vi "Scanning_ESR.vi"() -> ()   [LabVIEW 2024]
panel:
  out "Direction Indicator":bool
  in  "Direction":bool
  out "Y Steps":i32
  out "Data 2":string[][](array[string])
  out "Unaveraged data 2":string[][](array[string])
  out "Data":string[][](array[string])
  out "Unaveraged data":string[][](array[string])
  in  "file path (use dialog) 2":path=path "C:/Users/Crawford Group/Desktop/Angelo/NMR/DATA/Unaveraged&TimeStamp.txt"
  in  "file path (use dialog)":path=path "C:/Users/Crawford Group/Desktop/Angelo/NMR/DATA/DATA.txt"
  out "error out 2":errorcluster
  out "error out":errorcluster
  in  "Up?":bool
  out "Number of X":i32
  in  "Step size mm  Y":dbl=0.0017
  in  "Y Motor":refnum<k7>(container)
  in  "Step size mm X":dbl=0.0098
  in  "X Motor":refnum<k7>(container)
  in  "Number of X steps":dbl=1.0
  in  "Sweeps?":i32=1
  # "Averaged"
  # "Unaveraged"
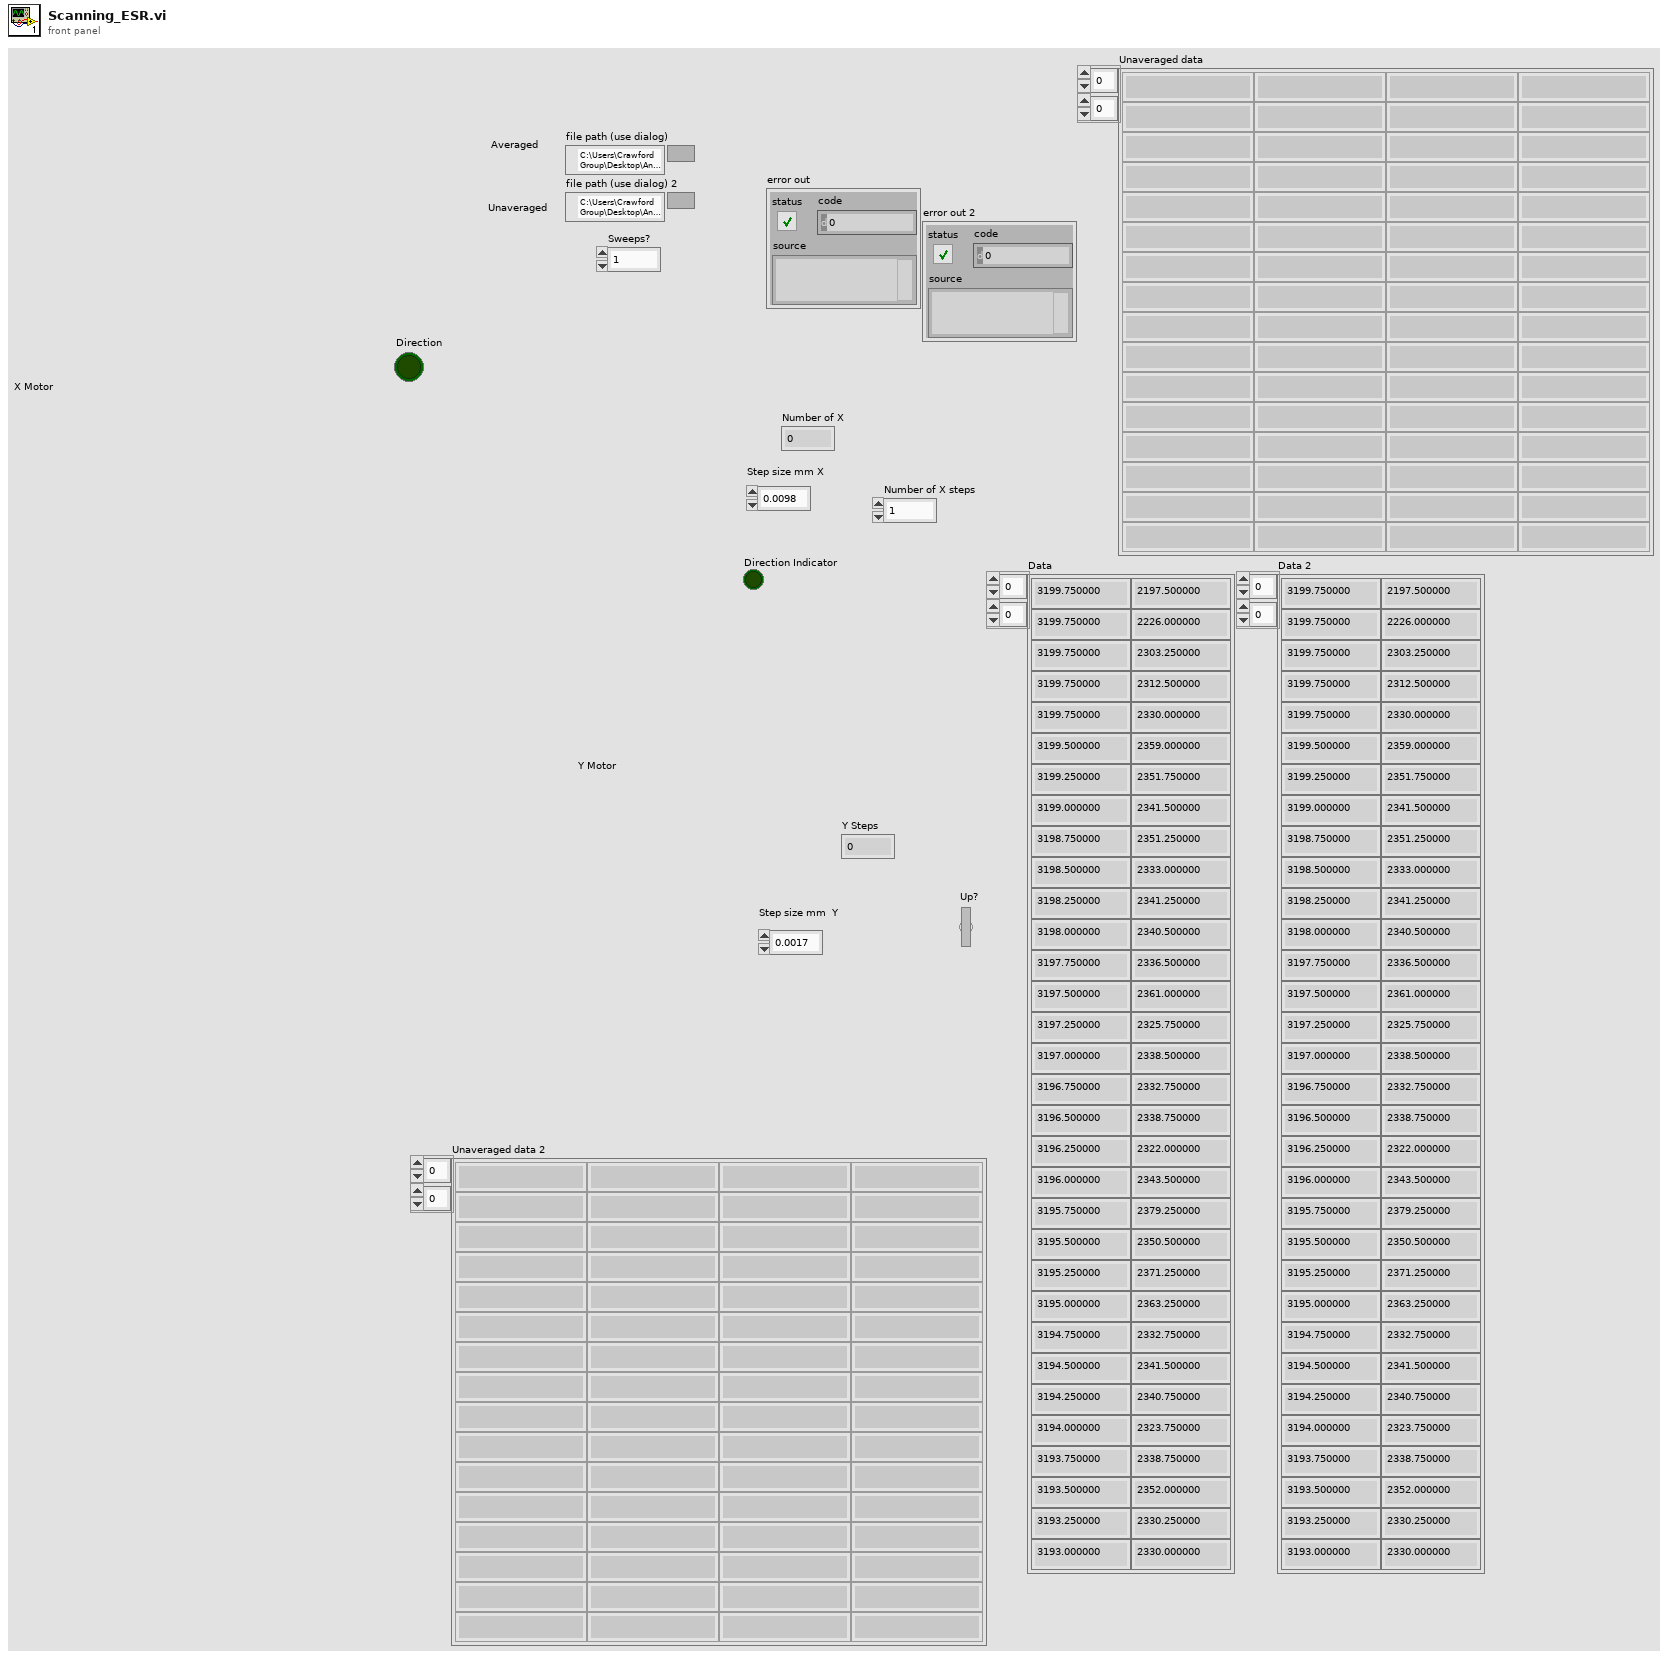
[diagram p1: front panel]
types:
  T1 = enum16{"open", "replace", "create", "open or create", "replace or create", "replace or create with confirmation"}
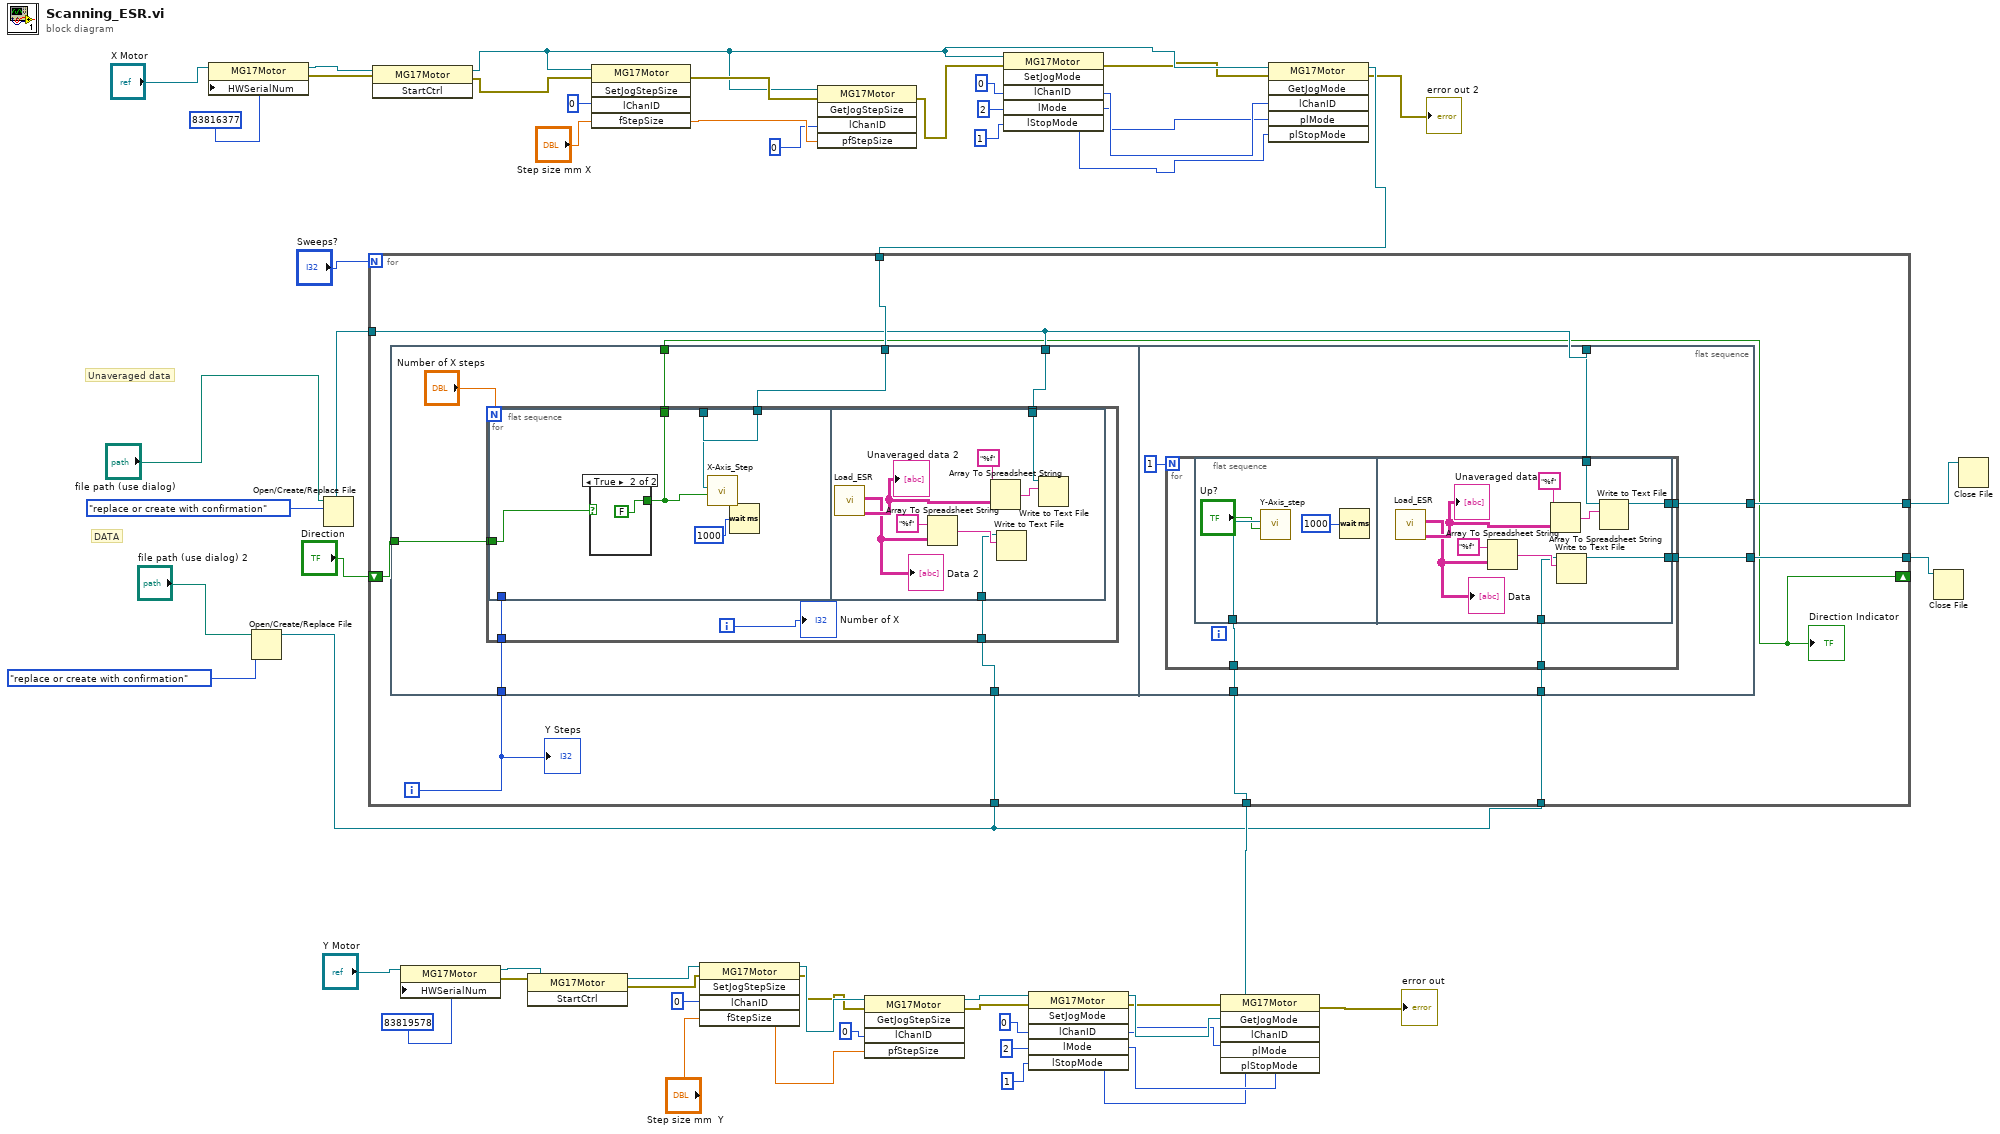
[diagram p0: block diagram]
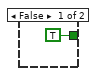
[diagram p2: hidden frame]
diagram:
  # "Unaveraged data"
  # "DATA"
  n1 = property class="MG17Motor"(reference="X Motor", "HWSerialNum"=83816377) -> (reference out=w54:refnum<k7>, error out=w53:errorcluster)  [unwired: 1 in]
  n2 = Open/Create/Replace File(file path (use dialog)="file path (use dialog) 2", operation (0:open)=T1."replace or create with confirmation") -> (refnum out=w20:refnum<file>)  [unwired: 4 in, 2 out]
  n3 = Open/Create/Replace File(file path (use dialog)="file path (use dialog)", operation (0:open)=T1."replace or create with confirmation") -> (refnum out=w22:refnum<file>)  [unwired: 4 in, 2 out]
  n4 = invoke class="MG17Motor" method="StartCtrl"(reference=w54, error in=w53) -> (reference out=w48:refnum<k7>, error out=w52:errorcluster)  [unwired: 1 in, 1 out]
  n5 = property class="MG17Motor"(reference="Y Motor", "HWSerialNum"=83819578) -> (reference out=w43:refnum<k7>, error out=w42:errorcluster)  [unwired: 1 in]
  n6 = invoke class="MG17Motor" method="StartCtrl"(reference=w43, error in=w42) -> (reference out=w41:refnum<k7>, error out=w40:errorcluster)  [unwired: 1 in, 1 out]
  n7 = invoke class="MG17Motor" method="SetJogStepSize"(reference=w48, error in=w52, "lChanID"=0, "fStepSize"="Step size mm X") -> (error out=w51:errorcluster, "fStepSize"=w50:sgl)  [unwired: 1 in, 3 out]
  n8 = invoke class="MG17Motor" method="SetJogStepSize"(reference=w41, error in=w40, "lChanID"=0, "fStepSize"="Step size mm  Y") -> (reference out=w39:refnum<k7>, error out=w38:errorcluster, "fStepSize"=w37:sgl)  [unwired: 1 in, 2 out]
  n9 = invoke class="MG17Motor" method="GetJogStepSize"(reference=w48, error in=w51, "lChanID"=0, "pfStepSize"=w50) -> (error out=w49:errorcluster)  [unwired: 1 in, 4 out]
  n10 = invoke class="MG17Motor" method="GetJogStepSize"(reference=w39, error in=w38, "lChanID"=0, "pfStepSize"=w37) -> (reference out=w36:refnum<k7>, error out=w35:errorcluster)  [unwired: 1 in, 3 out]
  n11 = invoke class="MG17Motor" method="SetJogMode"(reference=w48, error in=w49, "lChanID"=0, "lMode"=2, "lStopMode"=1) -> (error out=w47:errorcluster, "lChanID"=w46:i32, "lMode"=w45:i32, "lStopMode"=w28:i32)  [unwired: 1 in, 2 out]
  n12 = invoke class="MG17Motor" method="SetJogMode"(reference=w36, error in=w35, "lChanID"=0, "lMode"=2, "lStopMode"=1) -> (reference out=w34:refnum<k7>, error out=w33:errorcluster, "lChanID"=w32:i32, "lMode"=w31:i32, "lStopMode"=w30:i32)  [unwired: 1 in, 1 out]
  n13 = invoke class="MG17Motor" method="GetJogMode"(reference=w34, error in=w33, "lChanID"=w32, "plMode"=w31, "plStopMode"=w30) -> (reference out=w29:refnum<k7>, error out=→"error out":errorcluster)  [unwired: 1 in, 4 out]
  n14 = invoke class="MG17Motor" method="GetJogMode"(reference=w48, error in=w47, "lChanID"=w46, "plMode"=w45, "plStopMode"=w28) -> (reference out=w44:refnum<k7>, error out=→"error out 2":errorcluster)  [unwired: 1 in, 4 out]
  n15 = for {
    N: "Sweeps?" -> [_]
    tunnel: w29 -> [w65]
    tunnel: w44 -> [w64]
    tunnel: [w63] -> w23
    tunnel: w22 -> [w60]
    tunnel: w20 -> [w62]
    tunnel: [w61] -> w21
    tunnel: w20 -> [w59]
    shift-right: [w56] -> _
    shift-left: "Direction" -> [w57]
    i -> [w58]
    n16 = flat-sequence {
      tunnel: w64 -> [w71]
      tunnel: w60 -> [w70]
      tunnel: w59 -> [w69]
      tunnel: w58 -> [w68]
      tunnel: w57 -> [w67]
      tunnel: [w66] -> w56
      tunnel: w65 -> [w99]
      tunnel: [w98] -> w63
      tunnel: w60 -> [w97]
      tunnel: w62 -> [w96]
      tunnel: [w95] -> w61
      frame #0 {
        n17 = for {
          N: "Number of X steps" -> [_]
          tunnel: w71 -> [w78]
          tunnel: w70 -> [w77]
          tunnel: w69 -> [w76]
          tunnel: w68 -> [w75]
          tunnel: w67 -> [w74]
          tunnel: [w73] -> w66
          i -> [w79]
          n18 = flat-sequence {
            tunnel: w78 -> [w82]
            tunnel: w75 -> [_]
            tunnel: w74 -> [w81]
            tunnel: [w80] -> w73
            tunnel: w77 -> [w87]
            tunnel: w76 -> [w86]
            frame #0 {
              n19 = case shown="True" w81 {
                tunnel: [TRUE ("Left?") FALSE ("Left?")] -> w80
                frame False {
                }
                frame True {
                }
              }
              n20 = call "X-Axis_Step.vi"("Left?"=w80, "X Motor"=w82) -> ()  [unwired: 10 in]
              n21 = Wait (ms)(milliseconds to wait=u32 1000) -> ()  [unwired: 1 out]
            }
            frame #1 {
              n22 = call "Load_ESR.vi"() -> ("Unaveraged data"=w91:string[][], "Data"=w89:string[][])  [unwired: 9 in, 1 out]
              "Unaveraged data 2" <- w91
              "Data 2" <- w89
              n23 = Array To Spreadsheet String(array=w89, 3:"%f" ("format string")) -> (spreadsheet string=w88:string)  [unwired: 1 in]
              n24 = Array To Spreadsheet String(array=w91, 3:"%f" ("format string")) -> (spreadsheet string=w93:string)  [unwired: 1 in]
              n25 = Write to Text File(file (use dialog)=w86, text=w88) -> ()  [unwired: 2 in, 3 out]
              n26 = Write to Text File(file (use dialog)=w87, text=w93) -> ()  [unwired: 2 in, 3 out]
            }
          }
          "Number of X" <- w79
        }
      }
      frame #1 {
        n27 = for {
          N: 1 -> [_]
          tunnel: w99 -> [w104]
          tunnel: [w103] -> w98
          tunnel: w97 -> [w102]
          tunnel: w96 -> [w101]
          tunnel: [w100] -> w95
          n28 = flat-sequence {
            tunnel: w104 -> [w106]
            tunnel: [w114] -> w103
            tunnel: w102 -> [w113]
            tunnel: w101 -> [w109]
            tunnel: [w108] -> w100
            frame #0 {
              n29 = call "Y-Axis_step.vi"("Up?"="Up?", "Y Motor"=w106) -> ()  [unwired: 9 in, 1 out]
              n30 = Wait (ms)(milliseconds to wait=u32 1000) -> ()  [unwired: 1 out]
            }
            frame #1 {
              n31 = call "Load_ESR.vi"() -> ("Unaveraged data"=w115:string[][], "Data"=w111:string[][])  [unwired: 9 in, 1 out]
              "Unaveraged data" <- w115
              "Data" <- w111
              n32 = Array To Spreadsheet String(array=w111, 3:"%f" ("format string")) -> (spreadsheet string=w110:string)  [unwired: 1 in]
              n33 = Array To Spreadsheet String(array=w115, 3:"%f" ("format string")) -> (spreadsheet string=w117:string)  [unwired: 1 in]
              n34 = Write to Text File(file (use dialog)=w109, text=w110) -> (refnum out=w108:refnum<file>)  [unwired: 2 in, 2 out]
              n35 = Write to Text File(file (use dialog)=w113, text=w117) -> (refnum out=w114:refnum<file>)  [unwired: 2 in, 2 out]
            }
          }
        }
      }
    }
    "Y Steps" <- w58
    "Direction Indicator" <- w56
  }
  n36 = Close File(refnum=w21) -> ()  [unwired: 1 in, 2 out]
  n37 = Close File(refnum=w23) -> ()  [unwired: 1 in, 2 out]
